vi "Subpanel.vi"(8 "error in (no error)":errorcluster, 10 "String":string, 11 "Path":path) -> (0 "error out":errorcluster, 2 "Numeric":dbl, 3 "dup Path out":path)   [LabVIEW 2020]
doc: "Would be really cool if this worked!"
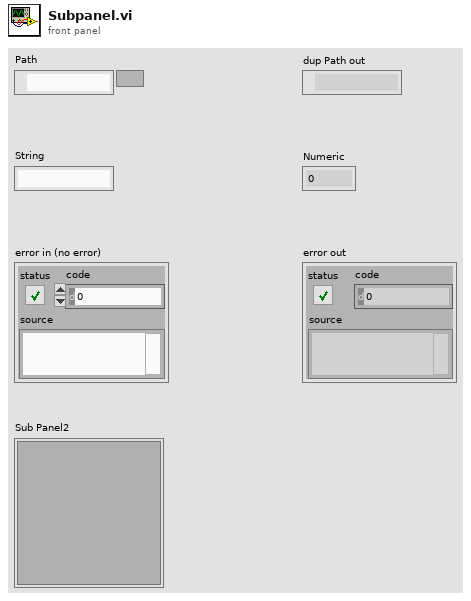
[diagram p1: front panel]
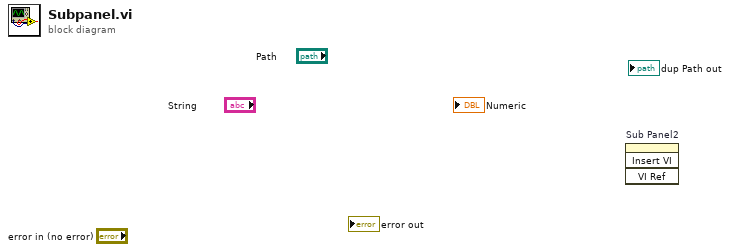
[diagram p0: block diagram]
diagram:
  n1 = invoke on="Sub Panel2" class="SubPnl" method="Insert VI"() -> ()  [unwired: 4 in, 4 out]
